vi "Rename project file.vi"(11 "Test Case In":refnum<class "Runner Unit Test - Prepare Project.lvclass">) -> (0 "error out":errorcluster, 3 "Test Case Out":refnum<class "Runner Unit Test - Prepare Project.lvclass">)   [LabVIEW 2026, in "Runner Unit Test - Prepare Project.lvclass"]
uses:
  Runner Unit Test - Prepare Project.lvclass
  C:/Program Files/National Instruments/LabVIEW 2026/vi.lib/Astemes/LUnit/Test Case.lvclass
  Actors/Runner/Runner/Runner.lvclass
  Interfaces/IRunner/IRunner/Interfaces--cluster.ctl
  Interfaces/IProject Manager/IProject Manager.lvclass
  Interfaces/IFile Manager/IFile Manager.lvclass
  Interfaces/IPython Caller/IPython Caller.lvclass
  Interfaces/IElement Manager/IElement Manager.lvclass
  Interfaces/ILV File Creator/ILV File Creator.lvclass
  Interfaces/IHash Whitelist Handler/IHash Whitelist Handler.lvclass
  Actors/Mock Logger/Mock Logger/Mock Logger.lvclass
  C:/Program Files/National Instruments/LabVIEW 2026/vi.lib/ActorFramework/Actor/Actor.lvclass
  <vilib>/ActorFramework/Message Enqueuer/Message Enqueuer.lvclass/Message Enqueuer.ctl
  <vilib>/ActorFramework/Message Enqueuer/Enqueue.vi
  Mocks/Mock IFile Manager/Mock IFile Manager.lvclass
  C:/Program Files/National Instruments/LabVIEW 2026/vi.lib/Astemes/LMock/Mock.lvclass
  C:/Users/juanj/Documents/hasbun_wood_engineering/github/py2vi/labview/Interfaces/IFile Manager/IFile Manager.lvclass
  <vilib>/ActorFramework/Stop Msg/Stop Msg.lvclass
  C:/Program Files/National Instruments/LabVIEW 2026/vi.lib/ActorFramework/Message/Message.lvclass
  <vilib>/Astemes/LMock/One Identical Inputs.vi
  <vilib>/ActorFramework/Message Priority Queue/Priority Enqueue.vi
  C:/Users/juanj/Documents/hasbun_wood_engineering/github/py2vi/labview/Mocks/Mock IFile Manager/Mock IFile Manager.lvclass
  Interfaces/IRunner/IRunner/IRunner.lvclass
  <vilib>/ActorFramework/Actor/Actor.lvclass
  <vilib>/Astemes/LMock/LMock Verifier.lvclass
  <vilib>/Astemes/LMock/LMock.lvlib
  <vilib>/Astemes/LMock/LMock One.lvlib
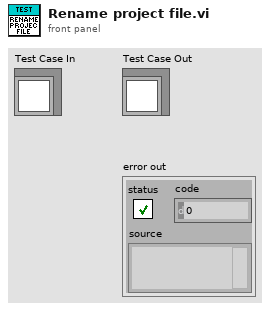
[diagram p1: front panel]
types:
  T1 = typedef "IRunner.lvlib/IRunner.lvclass/Interfaces--cluster.ctl" = cluster{"IProject Manager":refnum<class "IProject Manager.lvclass">, "IFile Manager":refnum<class "IFile Manager.lvclass">, "IPython Caller":refnum<class "IPython Caller.lvclass">, "IElement Manager":refnum<class "IElement Manager.lvclass">, "ILV File Creator":refnum<class "ILV File Creator.lvclass">, "IHash Whitelist Handler":refnum<class "IHash Whitelist Handler.lvclass">}
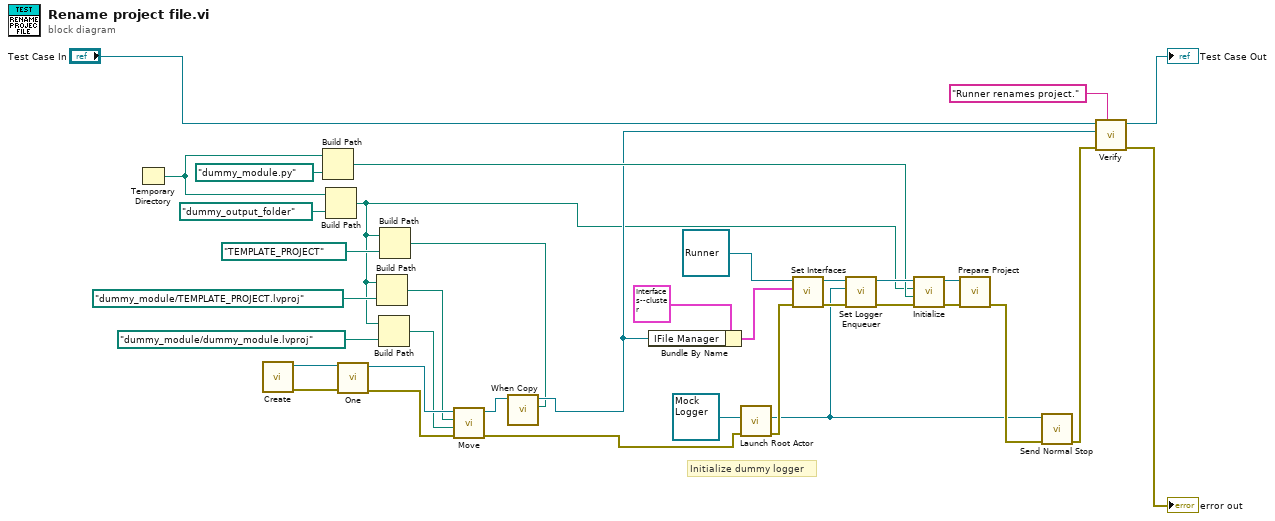
[diagram p0: block diagram]
diagram:
  # "Initialize dummy logger"
  n1 = Temporary Directory() -> (w12:path)
  n2 = call "Create.vi"() -> ("error out"=w35:errorcluster, "Mock Class Generator out"=w22:refnum<class "Mock IFile Manager.lvclass">)  [unwired: 10 in]
  n3 = Build Path(base path=w12, name or relative path=path "dummy_module.py") -> (appended path=w14:path)
  n4 = Build Path(base path=w12, name or relative path=path "dummy_output_folder") -> (appended path=w2:path)
  n5 = call-poly <vilib>:"One.vi"("error in (no error)"=w35, "Mock in"=w22) -> ("error out"=w29:errorcluster, "Mock out"=w13:refnum<class "Mock IFile Manager.lvclass">)  [unwired: 8 in]
  n6 = Build Path(base path=w2, name or relative path=path "dummy_module/TEMPLATE_PROJECT.lvproj") -> (appended path=w1:path)
  n7 = Build Path(base path=w2, name or relative path=path "dummy_module/dummy_module.lvproj") -> (appended path=w10:path)
  n8 = Build Path(base path=w2, name or relative path=path "TEMPLATE_PROJECT") -> (appended path=w6:path)
  n9 = call-dynamic "Move.vi"("error in"=w29, "Target"=w10, "Source"=w1, "IFile Manager in"=w13) -> ("error out"=w28:errorcluster, "IFile Manager out"=w8:refnum<class "Mock IFile Manager.lvclass">)  [unwired: 6 in]
  n10 = call "When Copy.vi"("New Path"=w6, "IFile Manager in"=w8) -> ("IFile Manager out"=w7:refnum<class "Mock IFile Manager.lvclass">)  [unwired: 9 in]
  n11 = Bundle By Name(cluster=T1 {"IProject Manager"=refnum, "IFile Manager"=refnum, "IPython Caller"=refnum, "IElement Manager"=refnum, "ILV File Creator"=refnum, "IHash Whitelist Handler"=refnum} ("Interfaces"), "IFile Manager"=w7) -> (w23:T1)
  n12 = call <vilib>:"Launch Root Actor.vi"("error in (no error)"=w28, "Actor"=refnum<class "Mock Logger.lvclass"> refnum ("Mock Logger.lvlib:Mock Logger.lvclass")) -> ("error out"=w34:errorcluster, "Actor's Enqueuer"=w20:refnum<class "Message Enqueuer.lvclass">)  [unwired: 8 in]
  n13 = call-dynamic "Set Interfaces.vi"("error in"=w34, "Interfaces"=w23, "Runner in"=refnum<class "Runner.lvclass"> refnum ("Runner.lvlib:Runner.lvclass")) -> ("error out"=w36:errorcluster, "Runner out"=w25:refnum<class "Runner.lvclass">)  [unwired: 7 in]
  n14 = call-dynamic "Set Logger Enqueuer.vi"("error in"=w36, "Logger"=w20, "Runner in"=w25) -> ("error out"=w31:errorcluster, "Runner out"=w17:refnum<class "Runner.lvclass">)  [unwired: 7 in]
  n15 = call-dynamic "Initialize.vi"("error in"=w31, "Python Module"=w14, "Output Folder"=w2, "G-CLI Runner in"=w17) -> ("error out"=w30:errorcluster, "G-CLI Runner out"=w16:refnum<class "Runner.lvclass">)  [unwired: 6 in]
  n16 = call-dynamic "Prepare Project.vi"("error in"=w30, "G-CLI Runner in"=w16) -> ("error out"=w33:errorcluster)  [unwired: 8 in, 1 out]
  n17 = call <vilib>:"Send Normal Stop.vi"("error in (no error)"=w33, "Message Enqueuer"=w20) -> ("error out"=w32:errorcluster)  [unwired: 9 in]
  n18 = call <vilib>:"Verify.vi"("Description"="Runner renames project.", "error in (no error)"=w32, "Mock"=w7, "LUnit Test Case In"="Test Case In") -> ("error out"=→"error out":errorcluster, "LUnit Test Case Out"=→"Test Case Out":refnum<class "Runner Unit Test - Prepare Project.lvclass">)  [unwired: 6 in]
